vi "create.from_cluster_pairs.vi"(10 "properties":cluster{"name":string, "value":string}[](array[cluster])) -> (3 "properties out":refnum<class "properties.lvclass">)   [LabVIEW 2020, in "nominal types.lvlib" / "properties.lvclass"]
uses:
  properties.lvclass
  properties.lvclass/properties.ctl
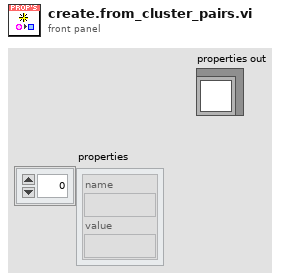
[diagram p1: front panel]
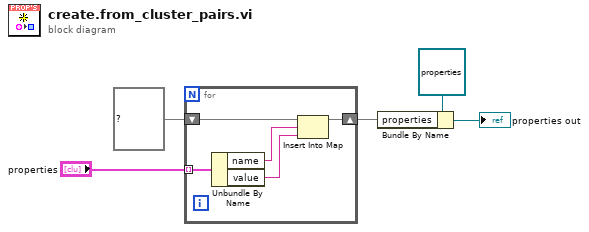
[diagram p0: block diagram]
diagram:
  n1 = for {
    shift-right: [w6] -> w2
    shift-left: map{string, string} {} ("properties") -> [w9]
    tunnel: "properties" -> [w10] mode=indexing
    n2 = Unbundle By Name(w10) -> ("name"=w8:string, "value"=w7:string)
    n3 = Insert Into Map(map in=w9, key=w8, value=w7) -> (map out=w6:map{string, string})  [unwired: 2 out]
  }
  n4 = Bundle By Name(cluster=refnum<class "properties.lvclass"> refnum ("properties out"), "properties"=w2) -> (→"properties out":refnum<class "properties.lvclass">)
